vi "Send Packet.vi"(6 "timeout (0ms : no ack)":i32, 8 "error in (no error)":errorcluster, 10 "Packet":refnum<class "ControlPacket.lvclass">, 11 "Session":refnum<class "Session.Client.lvclass">) -> (0 "error out":errorcluster, 1 "validated":bool, 2 "Response":refnum<class "ControlPacket.lvclass">[](array[class]), 3 "Session":refnum<class "Session.Client.lvclass">)   [LabVIEW 2013, in "MQTT Client.lvlib" / "Session.Client.lvclass"]
uses:
  Session.Client.lvclass
  <vilib>/LabVIEW Open Source Project/MQTT Control Packets/Control Packets/ControlPacket/ControlPacket.lvclass
  <vilib>/LabVIEW Open Source Project/MQTT Connection/MQTT_Base/Base Class/Response -- cluster.ctl
  <vilib>/LabVIEW Open Source Project/MQTT Connection/MQTT_Base/Session/Session.lvclass/Session.ctl
  <vilib>/LabVIEW Open Source Project/MQTT Connection/MQTT_Base/Base Class/MQTT_Base.lvclass
  <vilib>/LabVIEW Open Source Project/MQTT Connection/MQTT_Base/Session/Session.lvclass
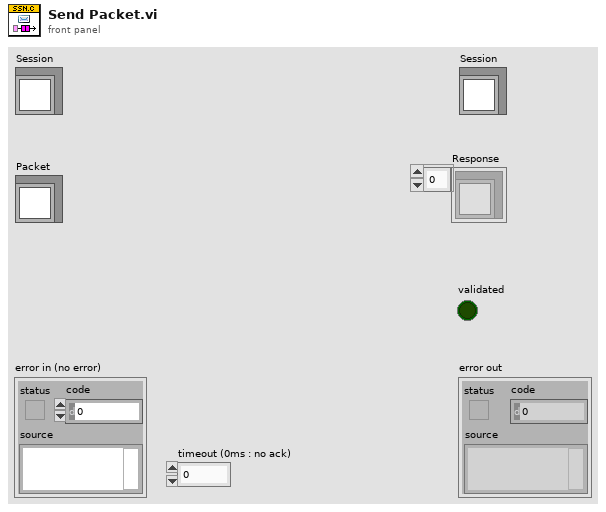
[diagram p1: front panel]
types:
  T1 = typedef "MQTT Base.lvlib/MQTT_Base.lvclass/Response -- cluster.ctl" = cluster{"Packet":refnum<class "ControlPacket.lvclass">, "Protocol Error":errorcluster, "disconnect session":bool, "[ACK]":refnum<notifier>[]}
  T2 = typedef "MQTT_Control_Packets.lvlib/ControlPacket.lvclass/Control Packet Type -- enum.ctl" = enum16{"Reserved", "CONNECT", "CONNACK", "PUBLISH", "PUBACK", "PUBREC", "PUBREL", "PUBCOMP", "SUBSCRIBE", "SUBACK", "UNSUBSCRIBE", "UNSUBACK", "PINGREQ", "PINGRESP", "DISCONNECT", "AUTH"}
  T3 = typedef "MQTT_Control_Packets.lvlib/ControlPacket.lvclass/QualityOfService -- enum.ctl" = enum16{"0 (At Most Once)", "1 (At Least Once)", "2 (Exactly Once)"}
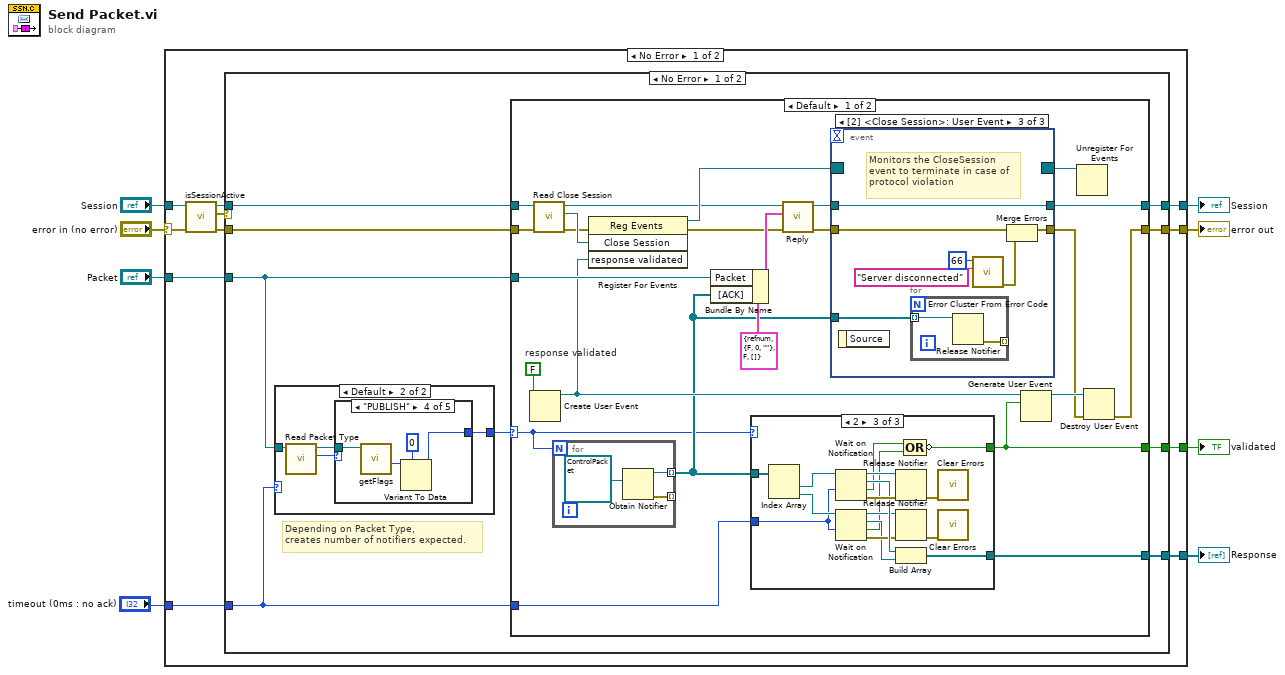
[diagram p0: block diagram]
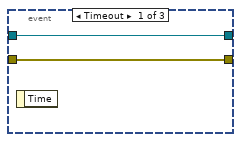
[diagram p2: hidden frame]
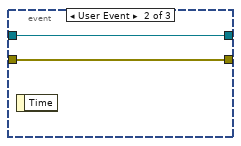
[diagram p3: hidden frame]
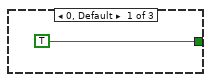
[diagram p4: hidden frame]
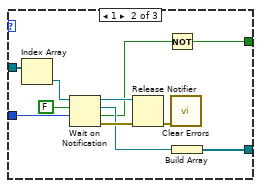
[diagram p5: hidden frame]
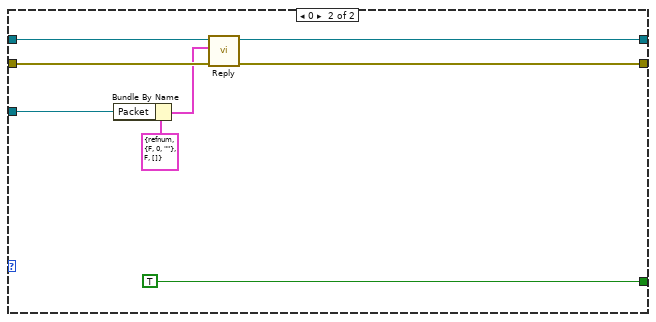
[diagram p6: hidden frame]
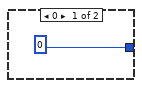
[diagram p7: hidden frame]
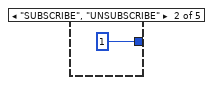
[diagram p9: hidden frame]
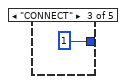
[diagram p10: hidden frame]
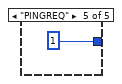
[diagram p11: hidden frame]
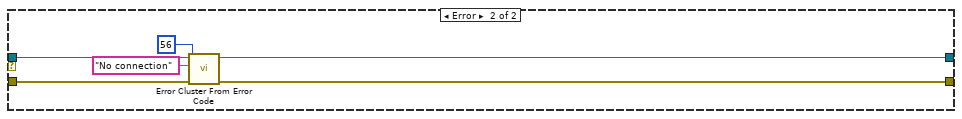
[diagram p12: hidden frame]
diagram:
  n1 = case shown="No Error" "error in (no error)" {
    selector: "error in (no error)" -> [w14 w122]
    tunnel: [w13 w122] -> w7
    tunnel: [w12 w121] -> w5
    tunnel: "Session" -> [w10 w121]
    tunnel: "Packet" -> [w18 _]
    tunnel: [w15 _] -> w3
    tunnel: "timeout (0ms : no ack)" -> [w17 _]
    tunnel: [w16 _] -> w1
    frame No Error {
      n2 = call <vilib>:"isSessionActive.vi"("Session in"=w10) -> ("error out"=w11:errorcluster, "Session out"=w9:refnum<class "Session.Client.lvclass">)  [unwired: 9 in]
      n3 = case shown="No Error" w11 {
        tunnel: w18 -> [w27 _]
        tunnel: w17 -> [w26 _]
        tunnel: [w25 _] -> w16
        tunnel: [w24 _] -> w15
        tunnel: w14 -> [w23 w117]
        tunnel: [w22 w116] -> w13
        tunnel: [w21 w120] -> w12
        tunnel: w9 -> [w19 w120]
        frame No Error {
          # "Depending on Packet Type, \ncreates number of notifiers expected."
          n4 = case shown="Default" w26 {
            tunnel: w27 -> [_ w108]
            tunnel: [0 w105] -> w20
            frame 0 {
            }
            frame Default {
              n5 = call <vilib>:"Read Packet Type.vi"("ControlPacket in"=w108) -> ("Control Packet Type"=w106:T2, "ControlPacket out"=w107:refnum<class "ControlPacket.lvclass">)  [unwired: 9 in]
              n6 = case shown="\"PUBLISH\"" w106 {
                tunnel: w107 -> [_ _ _ w113 _]
                tunnel: [_ 1 1 w112 1] -> w105
                frame Default {
                }
                frame "SUBSCRIBE", "UNSUBSCRIBE" {
                }
                frame "CONNECT" {
                }
                frame "PUBLISH" {
                  n7 = call-dynamic "getFlags.vi"("ControlPacket in"=w113) -> ("QoS"=w111:T3)  [unwired: 7 in, 3 out]
                  n8 = Variant To Data(type=0, Variant=w111) -> (data=w112:i32)  [unwired: 1 in, 1 out]
                }
                frame "PINGREQ" {
                }
              }
            }
          }
          n9 = case shown="Default" w20 {
            selector: w20 -> [w28 _]
            tunnel: w27 -> [w51 w103]
            tunnel: w19 -> [w34 w96]
            tunnel: w26 -> [w49 _]
            tunnel: [w48 _] -> w25
            tunnel: [w45 TRUE] -> w24
            tunnel: w23 -> [w32 w100]
            tunnel: [w41 w99] -> w22
            tunnel: [w30 w97] -> w21
            frame Default {
              w47 = FALSE  # response validated
              n10 = Create User Event(user event datatype=w47) -> (user event=w46:refnum<user-event>)  [unwired: 1 in, 1 out]
              n11 = call <vilib>:"Read Close Session.vi"("error in (no error)"=w32, "Session in"=w34) -> ("error out"=w31:errorcluster, "Close Session"=w35:refnum<user-event>, "Session out"=w33:refnum<class "Session.Client.lvclass">)  [unwired: 7 in]
              n12 = for {
                N: w28 -> [_]
                tunnel: [w95] -> _ mode=indexing
                tunnel: [w94] -> w39 mode=indexing
                n13 = Obtain Notifier(notification data type=refnum<class "ControlPacket.lvclass"> refnum ("Ack")) -> (notifier out=w94:refnum<notifier>, error out=w95:errorcluster)  [unwired: 3 in, 1 out]
              }
              n14 = register-events(error in=w31, w35, w46) -> (reference out=w44:refnum<event-registration>, error out=w37:errorcluster)  [unwired: 1 in]
              n15 = Bundle By Name(cluster=T1 {"Packet"=refnum, "Protocol Error"={"status"=FALSE, "code"=0, "source"=""}, "disconnect session"=FALSE, "[ACK]"=[]} ("element"), "Packet"=w51, "[ACK]"=w39) -> (w38:T1)
              n16 = case shown="2" w28 {
                tunnel: w49 -> [_ w76 w81]
                tunnel: w39 -> [_ w71 w89]
                tunnel: [_ w68 w87] -> w48
                tunnel: [TRUE w66 w78] -> w45
                frame 0, Default {
                }
                frame 1 {
                  n17 = Index Array(array=w71) -> (element=w70:refnum<notifier>)  [unwired: 1 in]
                  n18 = Wait on Notification(notifier=w70, ignore previous (F)=FALSE, timeout in ms (-1)=w76) -> (notifier out=w73:refnum<notifier>, notification=w72:refnum<class "ControlPacket.lvclass">, timed out?=w67:bool, error out=w74:errorcluster)  [unwired: 1 in]
                  n19 = Release Notifier(notifier=w73, error in (no error)=w74) -> (error out=w69:errorcluster)  [unwired: 1 in, 2 out]
                  n20 = Not(x=w67) -> (.not. x?=w66:bool)
                  n21 = call <vilib>:"Clear Errors.vi"("error in (no error)"=w69) -> ()  [unwired: 6 in, 1 out]
                  n22 = Build Array(w72) -> (w68:refnum<class "ControlPacket.lvclass">[])
                }
                frame 2 {
                  n23 = Index Array(array=w89) -> (element #1=w77:refnum<notifier>, element #2=w83:refnum<notifier>)  [unwired: 2 in]
                  n24 = Wait on Notification(notifier=w77, timeout in ms (-1)=w81) -> (notifier out=w91:refnum<notifier>, notification=w90:refnum<class "ControlPacket.lvclass">, timed out?=w80:bool, error out=w92:errorcluster)  [unwired: 2 in]
                  n25 = Wait on Notification(notifier=w83, timeout in ms (-1)=w81) -> (notifier out=w82:refnum<notifier>, notification=w84:refnum<class "ControlPacket.lvclass">, timed out?=w79:bool, error out=w85:errorcluster)  [unwired: 2 in]
                  n26 = Release Notifier(notifier=w91, error in (no error)=w92) -> (error out=w88:errorcluster)  [unwired: 1 in, 2 out]
                  n27 = Release Notifier(notifier=w82, error in (no error)=w85) -> (error out=w86:errorcluster)  [unwired: 1 in, 2 out]
                  n28 = Build Array(w90, w84) -> (w87:refnum<class "ControlPacket.lvclass">[])
                  n29 = Compound Arithmetic op=OR(w80, w79) -> (invert w78:bool)
                  n30 = call <vilib>:"Clear Errors.vi"("error in (no error)"=w88) -> ()  [unwired: 6 in, 1 out]
                  n31 = call <vilib>:"Clear Errors.vi"("error in (no error)"=w86) -> ()  [unwired: 6 in, 1 out]
                }
              }
              n32 = call <vilib>:"Reply.vi"("error in (no error)"=w37, "Outgoing Element"=w38, "Session in"=w33) -> ("error out"=w36:errorcluster, "Session out"=w29:refnum<class "Session.Client.lvclass">)  [unwired: 7 in]
              n33 = event shown="[2] <Close Session>: User Event" {
                selector: w44 -> [_ _ _]
                dyn-events: [_ _ _] -> w43
                timeout: _ -> [_ _ _]
                tunnel: w36 -> [w53 w55 w58]
                tunnel: [w53 w55 w59] -> w40
                tunnel: w39 -> [_ _ w62]
                tunnel: [w52 w54 w56] -> w30
                tunnel: w29 -> [w52 w54 w56]
                event Timeout {
                  n34 = event-data() -> ()  [unwired: 1 in, 1 out]
                }
                event User Event {
                  n35 = event-data() -> ()  [unwired: 1 in, 1 out]
                }
                event User Event {
                  # "Monitors the CloseSession\nevent to terminate in case of\nprotocol violation"
                  n36 = event-data() -> ()  [unwired: 1 in, 1 out]
                  n37 = for {
                    tunnel: w62 -> [w64] mode=indexing
                    tunnel: [w63] -> _ mode=indexing
                    n38 = Release Notifier(notifier=w64) -> (error out=w63:errorcluster)  [unwired: 2 in, 2 out]
                  }
                  n39 = call <vilib>:"Error Cluster From Error Code.vi"("error message (\"\")"="Server disconnected" ("error message (\"\")"), "error code (0)"=66) -> ("error out"=w57:errorcluster)  [unwired: 7 in]
                  n40 = Merge Errors(w58, w57) -> (w59:errorcluster)
                }
              }
              n41 = Generate User Event(user event=w46, event data cluster=w45) -> (user event out=w42:refnum<user-event>)  [unwired: 2 in, 1 out]
              n42 = Unregister For Events(event registration refnum=w43) -> ()  [unwired: 1 in, 1 out]
              n43 = Destroy User Event(user event=w42, error in=w40) -> (error out=w41:errorcluster)
            }
            frame 0 {
              n44 = Bundle By Name(cluster=T1 {"Packet"=refnum, "Protocol Error"={"status"=FALSE, "code"=0, "source"=""}, "disconnect session"=FALSE, "[ACK]"=[]} ("element"), "Packet"=w103) -> (w98:T1)
              n45 = call <vilib>:"Reply.vi"("error in (no error)"=w100, "Outgoing Element"=w98, "Session in"=w96) -> ("error out"=w99:errorcluster, "Session out"=w97:refnum<class "Session.Client.lvclass">)  [unwired: 7 in]
            }
          }
        }
        frame Error {
          n46 = call <vilib>:"Error Cluster From Error Code.vi"("error in (no error)"=w117, "error message (\"\")"="No connection" ("error message (\"\")"), "error code (0)"=56) -> ("error out"=w116:errorcluster)  [unwired: 6 in]
        }
      }
    }
    frame Error {
    }
  }
  "error out" <- w7
  "Session" <- w5
  "validated" <- w3
  "Response" <- w1
